vi "GT_Parse.vi"(11 "Words":u16[](array[numeric])) -> (3 "Status":T1)   [LabVIEW 2018]
doc: "Use this template to build a VI to use as a subVI."
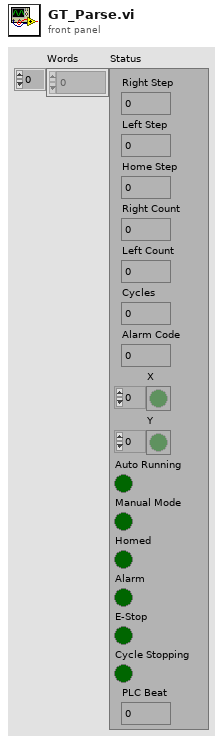
[diagram p1: front panel]
types:
  T1 = cluster{"Right Step":u16, "Left Step":u16, "Home Step":u16, "Right Count":u16, "Left Count":u16, "Cycles":u16, "Alarm Code":u16, "X":bool[], "Y":bool[], "Auto Running":bool, "Manual Mode":bool, "Homed":bool, "Alarm":bool, "E-Stop":bool, "Cycle Stopping":bool, "PLC Beat":u16}
  T2 = cluster{u16, u16, u16, u16, u16, u16, u16, "Boolean array":bool[], "Boolean array":bool[], bool, bool, bool, bool, bool, bool, u16}
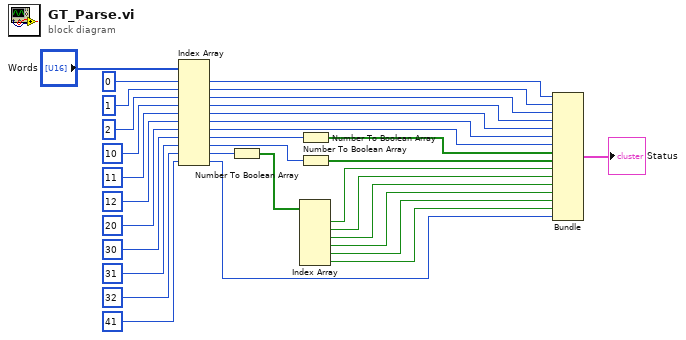
[diagram p0: block diagram]
diagram:
  n1 = Index Array(array="Words", index #1=0 ("index"), index #2=1 ("index"), index #3=2 ("index"), index #4=10 ("index"), index #5=11 ("index"), index #6=12 ("index"), index #7=20 ("index"), index #8=30 ("index"), index #9=31 ("index"), index #10=32 ("index"), index #11=41 ("index")) -> (element #1=w21:u16, element #2=w20:u16, element #3=w19:u16, element #4=w18:u16, element #5=w17:u16, element #6=w16:u16, element #7=w15:u16, element #8=w14:u16, element #9=w12:u16, element #10=w10:u16, element #11=w2:u16)
  n2 = Number To Boolean Array(number=w10) -> (Boolean array=w9:bool[])
  n3 = Index Array(array=w9) -> (element #1=w8:bool, element #2=w7:bool, element #3=w6:bool, element #4=w5:bool, element #5=w4:bool, element #6=w3:bool)  [unwired: 6 in]
  n4 = Number To Boolean Array(number=w14) -> (Boolean array=w13:bool[])
  n5 = Number To Boolean Array(number=w12) -> (Boolean array=w11:bool[])
  n6 = Bundle(w21, w20, w19, w18, w17, w16, w15, "Boolean array"=w13, "Boolean array"=w11, w8, w7, w6, w5, w4, w3, w2) -> (→"Status":T2)  [unwired: 1 in]
